vi "VIH ProjFile - Build Control Tag String.vi"(8 "error in":errorcluster, 9 "tag misses top control (T)":bool=TRUE, 11 "Ctl Refnum":refnum<vi>) -> (0 "error out":errorcluster, 1 "Control Class":string, 2 "Control Tag":string, 3 "dup Ctl Refnum":refnum<vi>, 5 "Label":string)   [LabVIEW 2014]
doc: "The VI builds a Control Tag of the specified control.\n\n::: VI Helpeks :::\nCopyright (c) 2000-2026 Konstantin Shifershteyn. All rights reserved."
panel:
  # "VI Helpeks\nCopyright (c) 2012-2026 Konstantin Shifershteyn"
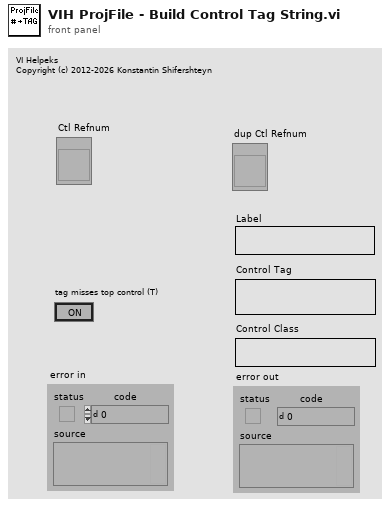
[diagram p1: front panel]
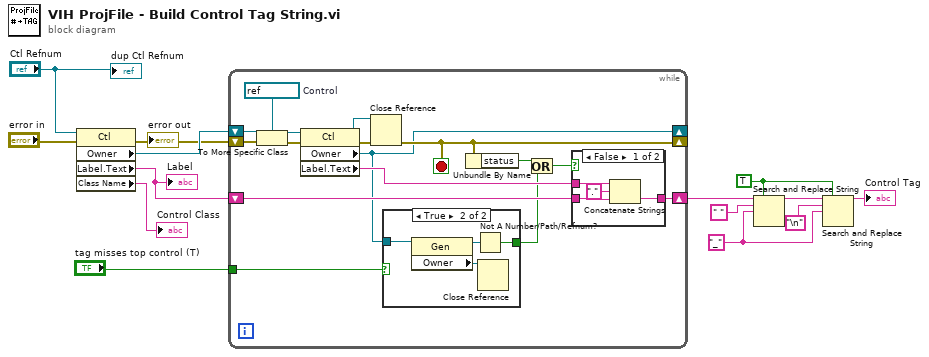
[diagram p0: block diagram]
diagram:
  w3 = "_" ("replace string (\"\")")
  w4 = TRUE
  n1 = property class="Ctl"(reference="Ctl Refnum", error in="error in") -> (error out=w11:errorcluster, "Owner"=w14:refnum<vi>, "Label.Text"=w9:string, "Class Name"=→"Control Class":string)  [unwired: 1 out]
  "error out" <- w11
  "Label" <- w9
  n2 = while {
    shift-right: [w25] -> _
    shift-left: w11 -> [w17]
    shift-right: [w26] -> w6
    shift-left: w9 -> [w28]
    shift-right: [w22] -> _
    shift-left: w14 -> [w18]
    tunnel: "tag misses top control (T)" -> [w20]
    stop <- w25 stop-if-true
    w19 = refnum<vi> refnum  # Control
    n3 = To More Specific Class(target class=w19, reference=w18, error in=w17) -> (specific class reference=w15:refnum<vi>, error out=w16:errorcluster)
    n4 = property class="Ctl"(reference=w15, error in=w16) -> (reference out=w30:refnum<vi>, error out=w29:errorcluster, "Owner"=w22:refnum<vi>, "Label.Text"=w27:string)
    n5 = Close Reference(reference=w30, error in (no error)=w29) -> (error out=w25:errorcluster)
    n6 = case shown="True" w20 {
      tunnel: w22 -> [_ w33]
      tunnel: [_ w31] -> w21
      frame False {
      }
      frame True {
        n7 = property class="Gen"(reference=w33) -> ("Owner"=w32:refnum<vi>)  [unwired: 1 in, 2 out]
        n8 = Not A Number/Path/Refnum?(number/path/refnum=w32) -> (NaN/Path/Refnum?=w31:bool)
        n9 = Close Reference(reference=w32) -> ()  [unwired: 1 in, 1 out]
      }
    }
    n10 = Unbundle By Name(w25) -> ("status"=w24:bool)
    n11 = Or(x=w24, y=w21) -> (x .or. y?=w23:bool)
    n12 = case shown="False" w23 {
      tunnel: w28 -> [w37 w38]
      tunnel: w27 -> [w36 _]
      tunnel: [w34 w38] -> w26
      frame False {
        n13 = Concatenate Strings(w36, "." ("string"), w37) -> (w34:string)
      }
      frame True {
      }
    }
  }
  n14 = Search and Replace String(replace all?=w4, input string=w6, search string=" ", replace string=w3) -> (result string=w5:string)  [unwired: 4 in, 3 out]
  n15 = Search and Replace String(replace all?=w4, input string=w5, search string="\n", replace string=w3) -> (result string=→"Control Tag":string)  [unwired: 4 in, 3 out]
  "dup Ctl Refnum" <- "Ctl Refnum"
